vi "Python TCP Connection Handler.vi"(9 "Additional Data":variant, 10 "connection ID":T1, 11 "TCP Server Refnum":refnum<class "JKI TCP Server.lvclass">) -> ()   [LabVIEW 2020, in "jki_python_bridge.lvlib" / "Server.lvclass"]
uses:
  Server.lvclass
  <vilib>/addons/_JKI.lib/_JKI_lib_TCP_Server.llb/TCP Server Connection Session ID Cluster.ctl
  <vilib>/addons/_JKI.lib/_JKI_lib_TCP_Server.llb/JKI TCP Server.lvclass
  Type Definitions/PythonResponseType.ctl
  Type Definitions/Python Class Data - Cluster.ctl
  PyObject/PyObject.lvclass/PyObject.ctl
  Python Data Tools/source/LabVIEW Data to Python String/LabVIEW Data to Python String (String).vi
  Python Data Tools/source/LabVIEW Data to Python String/LabVIEW Data to Python String (Variant).vi
  Server.lvclass/Server.ctl
  PyObject/PyObject.lvclass
  Python Data Tools/source/jki_python_data_tools.lvlib
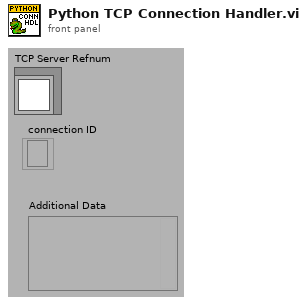
[diagram p1: front panel]
types:
  T1 = typedef "JKI TCP Server.lvclass/TCP Server Connection Session ID Cluster.ctl" = refnum<k5>
  T2 = enum16{"Standard", "Buffered", "CRLF", "Immediate"}
  T3 = typedef "jki_python_bridge.lvlib/Server.lvclass/PythonResponseType.ctl" = enum16{"ERRor", "OK", "NEXT"}
  T4 = typedef "jki_python_bridge.lvlib/Server.lvclass/Python Class Data - Cluster.ctl" = cluster{"Name":string, "Functions":cluster{"Name":string, "Arguments":string[], "Documentation":string}[]}
  T5 = typedef "jki_python_bridge.lvlib/Server.lvclass/Python Node.ctl" = cluster{"Name":string, "Python Method Call":refnum<user-event>, "Call Handle":refnum<class "PyObject.lvclass">}
  T6 = cluster{"Name":string, "Arguments":string[], "Documentation":string}[]
  T7 = typedef "jki_python_bridge.lvlib/Server.lvclass/Python Response - Cluster.ctl" = cluster{"Python Response":variant, "error out":errorcluster}
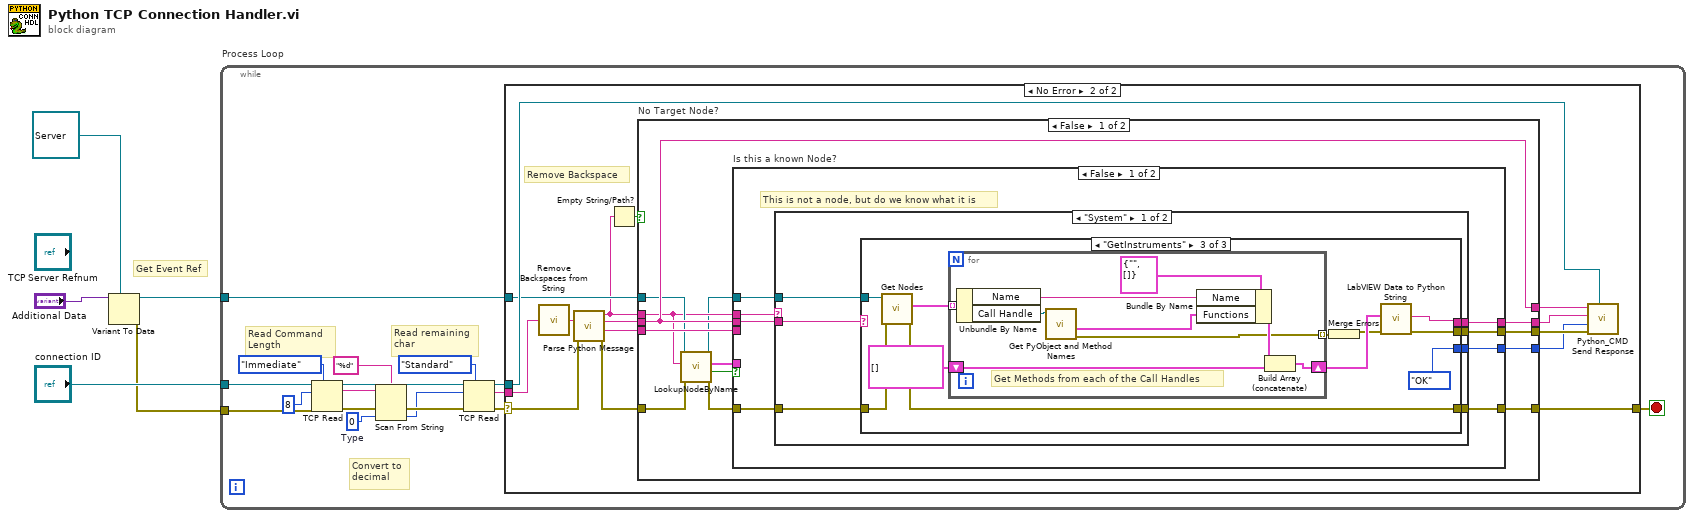
[diagram p0: block diagram]
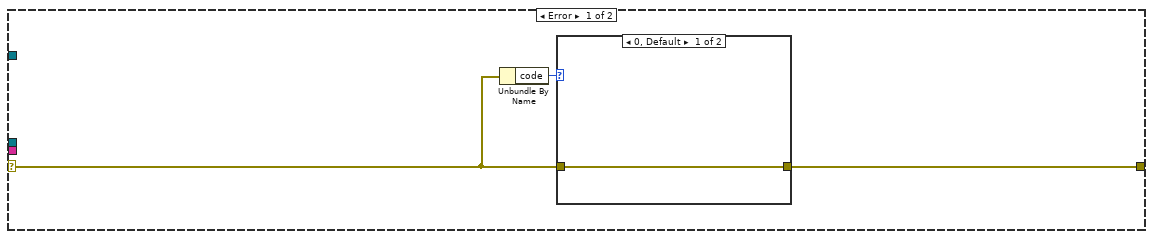
[diagram p2: hidden frame]
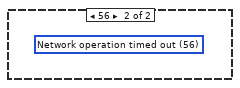
[diagram p3: hidden frame]
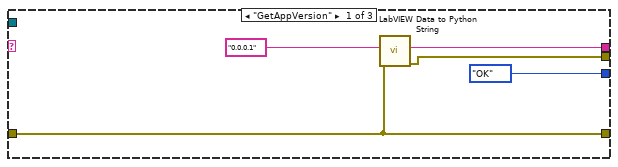
[diagram p4: hidden frame]
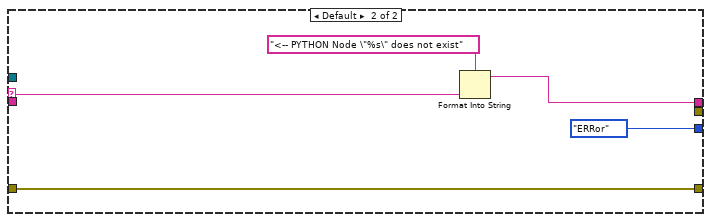
[diagram p6: hidden frame]
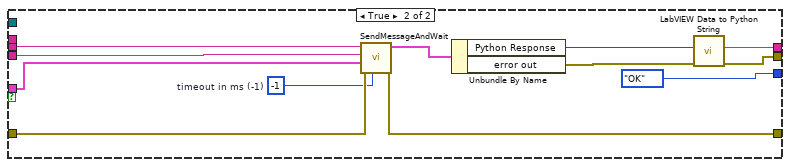
[diagram p7: hidden frame]
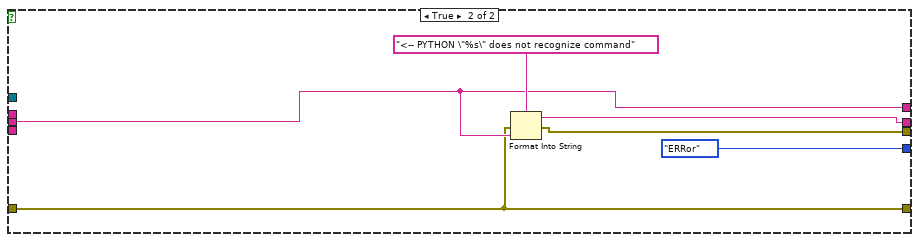
[diagram p8: hidden frame]
diagram:
  # "Get Event Ref"
  n1 = Variant To Data(type=refnum<class "Server.lvclass"> refnum ("JKI_Python_Server in"), Variant="Additional Data") -> (data=w2:refnum<class "Server.lvclass">, error out=w1:errorcluster)  [unwired: 1 in]
  n2 = while "Process Loop" {
    tunnel: "connection ID" -> [w17]
    tunnel: w2 -> [w7]
    tunnel: w1 -> [w6]
    stop <- w22 stop-if-true
    w9 = 0  # Type
    # "Read remaining\nchar"
    # "Convert to\ndecimal"
    # "Read Command\nLength"
    n3 = TCP Read(connection ID=w17, bytes to read=8, error in (no error)=w6, 7:T2."Immediate" ("mode (standard)")) -> (connection ID out=w16:T1, data out=w13:string, error out=w14:errorcluster)  [unwired: 1 out]
    n4 = Scan From String(format string="%d", input string=w13, error in=w14, default 1=w9) -> (error out=w12:errorcluster, output 1=w8:i32)  [unwired: 1 in, 2 out]
    n5 = TCP Read(connection ID=w16, bytes to read=w8, error in (no error)=w12, 7:T2."Standard" ("mode (standard)")) -> (connection ID out=w18:T1, data out=w19:string, error out=w20:errorcluster)  [unwired: 1 out]
    n6 = case shown="No Error" w20 {
      selector: w20 -> [w24 w30]
      tunnel: w18 -> [_ w33]
      tunnel: w19 -> [_ w28]
      tunnel: [w23 w41] -> w22
      tunnel: w7 -> [_ w32]
      frame Error {
        n7 = Unbundle By Name(w24) -> ("code"=w25:i32)
        n8 = case shown="0, Default" w25 {
          tunnel: w24 -> [w26 _]
          tunnel: [w26 _] -> w23
          frame 0, Default {
          }
          frame 56 {
            (unwired) 56 items=["No error", "Argument error", "Memory is full", "Out of zone", "End of file", "File already open", "Generic file I/O error", "File not found", "File permission error", "Disk is full", "Duplicate path", "Too many files open", "System feature not enabled", "Resource file not found", "Cannot add resource", "Resource not found", "Image not found", "Image memory error", "Pen does not exist", "Config type invalid", "Config token not found", "Config parse error", "Config memory error", "Bad external code format", "Bad external code offset", "External code not present", "Null window", "Destroy window error", "Null menu", "Print aborted", "Bad print record", "Print driver error", "Windows error during printing", "Memory error during printing", "Print dialog error", "Generic print error", "Invalid device refnum", "Device not found", "Device parameter error", "Device unit error", "Cannot open device", "Device call aborted", "Generic error", "Cancelled by user", "Object ID too low", "Object ID too high", "Object not in heap", "Unknown heap", "Unknown object (invalid DefProc)", "Unknown object (DefProc not in table)", "Message out of range", "Invalid (null) method", "Unknown message", "Manager call not supported", "Bad address", "Network operation in progress", "Network operation timed out", "Connection is busy", "Network attribute not supported", "Network error", "Address in use", "System out of memory", "Connection aborted", "Connection refused", "Not connected", "Already connected", "Connection closed", "Initialization error (interapplication manager)", "Bad occurrence", "Wait on unbound occurrence handler", "Occurrence queue overflow", "Datalog type conflict", "Unused", "Unrecognized type (interapplication manager)", "Memory corrupt", "Failed to make temporary DLL", "Old CIN version", "Drag socket not found", "Failed to load drop-object", "Failed to register OLE object", "Failed to release OLE object", "Format specifier type mismatch", "Unknown format specifier", "Too few format specifiers", "Too many format specifiers", "Scan failed", "Newer CIN version", "Error converting to variant", "Runtime menu error", "Password tampered", "Variant attribute not found", "Incompatible variant data type", "Event data is not available", "Event Store is not present", "Occurrence is not found", "Event Queue is not created", "Event info is not available", "Refnum passed is NULL", "Error retrieving Class GUID", "Error retrieving CoClass GUID", "Error retrieving TypeLib GUID.", "Bad built application magic bytes.", "Specific driver is different from the specific driver associated with the Logical Name.", "There is no session opened to the class driver.", "Max Error", "MAX - Error with config objects", "MAX - Error loading configuration", "MAX - Group not supported"]
          }
        }
      }
      frame No Error {
        # "Remove Backspace"
        n9 = call "Remove Backspaces from String.vi"("String in"=w28) -> ("String out"=w27:string)  [unwired: 4 in]
        n10 = call "Parse Python Message.vi"("error in"=w30, "Python Message"=w27) -> ("error out"=w29:errorcluster, "Argument String"=w38:string, "PYTHON Command"=w39:string, "PYTHON Node Name"=w31:string)  [unwired: 6 out]
        n11 = Empty String/Path?(string/path=w31) -> (empty?=w37:bool)
        n12 = case "No Target Node?" shown="False" w37 {
          tunnel: [w54 w113] -> w41
          tunnel: [w53 w117] -> w40
          tunnel: w29 -> [w47 w113]
          tunnel: w39 -> [w51 w114]
          tunnel: w38 -> [w52 _]
          tunnel: [w49 w118] -> w36
          tunnel: [w51 w114] -> w35
          tunnel: [w50 PythonResponseType."ERRor" ("Response Type")] -> w34
          tunnel: w32 -> [w45 _]
          tunnel: w31 -> [w43 _]
          frame False {
            n13 = call "LookupNodeByName.vi"("error in (no error)"=w47, "Python Node Name"=w43, "Server in"=w45) -> ("error out"=w46:errorcluster, "Found?"=w48:bool, "PYTHON Node"=w44:T5, "Server out"=w42:refnum<class "Server.lvclass">)  [unwired: 5 in]
            n14 = case "Is this a known Node?" shown="False" w48 {
              tunnel: [w57 w112] -> w54
              tunnel: [w60 w109] -> w53
              tunnel: w46 -> [w58 w108]
              tunnel: w52 -> [_ w107]
              tunnel: w51 -> [w61 w106]
              tunnel: [w59 PythonResponseType."OK" ("Response Type")] -> w50
              tunnel: [w55 w104] -> w49
              tunnel: w44 -> [_ w103]
              tunnel: w43 -> [w62 _]
              tunnel: w42 -> [w56 _]
              frame False {
                # "This is not a node, but do we know what it is"
                n15 = case shown="\"System\"" w62 {
                  selector: w62 -> [_ w98]
                  tunnel: w61 -> [w67 _]
                  tunnel: [w69 w100] -> w60
                  tunnel: [w66 PythonResponseType."ERRor" ("Response Type")] -> w59
                  tunnel: w58 -> [w65 w96]
                  tunnel: [w68 w96] -> w57
                  tunnel: w56 -> [w64 _]
                  tunnel: [w63 _] -> w55
                  frame "System" {
                    n16 = case shown="\"GetInstruments\"" w67 {
                      tunnel: [w72 _ w79] -> w69
                      tunnel: w65 -> [w70 w75 w84]
                      tunnel: [w70 w75 w78] -> w68
                      tunnel: [PythonResponseType."OK" ("Response Type") _ PythonResponseType."OK" ("Response Type")] -> w66
                      tunnel: w64 -> [_ _ w85]
                      tunnel: [w71 _ w81] -> w63
                      frame "GetAppVersion" {
                        n17 = call-poly "LabVIEW Data to Python String.vi"("error in (no error)"=w70, "LabVIEW Data"="0.0.0.1" ("Python String")) -> ("error out"=w71:errorcluster, "Python String"=w72:string)  [unwired: 8 in]
                      }
                      frame Default {
                      }
                      frame "GetInstruments" {
                        n18 = call "Get Nodes.vi"("error in (no error)"=w84, "JKI_Python_Server in"=w85) -> ("error out"=w78:errorcluster, "Nodes"=w83:T5[])  [unwired: 7 in, 1 out]
                        n19 = for {
                          tunnel: w83 -> [w95] mode=indexing
                          shift-right: [w94] -> w80
                          shift-left: T4[] [] -> [w93]
                          tunnel: [w88] -> w77 mode=indexing
                          # "Get Methods from each of the Call Handles"
                          n20 = Unbundle By Name(w95) -> ("Name"=w91:string, "Call Handle"=w92:refnum<class "PyObject.lvclass">)
                          n21 = call "Get PyObject and Method Names.vi"("Node in"=w92) -> ("error out"=w88:errorcluster, "Functions"=w87:T6)  [unwired: 7 in, 2 out]
                          n22 = Bundle By Name(cluster=T4 {"Name"="", "Functions"=[]} ("Python Class Data"), "Name"=w91, "Functions"=w87) -> (w89:T4)
                          n23 = Build Array (concatenate)(w89, w93) -> (w94:T4[])
                        }
                        n24 = Merge Errors(w77) -> (w76:errorcluster)
                        n25 = call-poly "LabVIEW Data to Python String.vi"("error in (no error)"=w76, "LabVIEW Data"=w80) -> ("error out"=w81:errorcluster, "Python String"=w79:string)  [unwired: 8 in]
                      }
                    }
                  }
                  frame Default {
                    n26 = Format Into String(format string="<-- PYTHON Node \"%s\" does not exist", w98) -> (resulting string=w100:string)  [unwired: 2 in, 1 out]
                  }
                }
              }
              frame True {
                w101 = -1  # timeout in ms (-1)
                n27 = call "SendMessageAndWait.vi"("timeout in ms (-1)"=w101, "error in (no error)"=w108, "PYTHON Node"=w103, "Argument String"=w107, "PYTHON Command"=w106) -> ("error out"=w112:errorcluster, "Reply"=w102:T7)  [unwired: 5 in]
                n28 = Unbundle By Name(w102) -> ("Python Response"=w110:variant, "error out"=w111:errorcluster)
                n29 = call-poly "LabVIEW Data to Python String.vi"("error in (no error)"=w111, "LabVIEW Data"=w110) -> ("error out"=w104:errorcluster, "Python String"=w109:string)  [unwired: 8 in]
              }
            }
          }
          frame True {
            n30 = Format Into String(format string="<-- PYTHON \"%s\" does not recognize command", error in=w113, w114) -> (resulting string=w117:string, error out=w118:errorcluster)  [unwired: 1 in]
          }
        }
        n31 = call "Python_CMD Send Response.vi"("TCP Connection ID"=w33, "non-fatal error"=w36, "Response Type"=w34, "Response"=w40, "PYTHON Command String"=w35) -> ()  [unwired: 6 in, 1 out]
      }
    }
  }
